vi "Convert and Enqueue.vi"(8 "error in":errorcluster, 10 "UI GUID":string, 11 "Data":u8[](array[numeric])) -> (0 "error out":errorcluster, 3 "Table Data":string[][](array[string]))   [LabVIEW 2025, in "CAN-LIN Raw Bus Capture UI.lvlib"]
uses:
  CAN-LIN Raw Bus Capture UI.lvlib
  Enqueue Data.vi
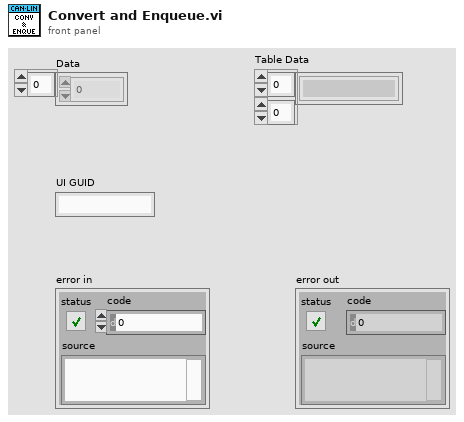
[diagram p1: front panel]
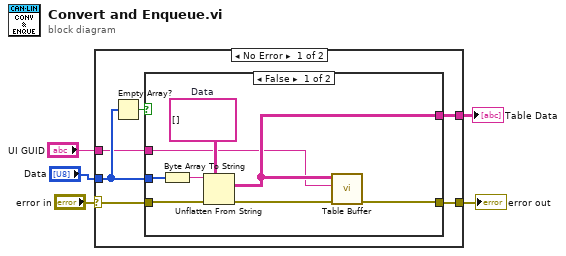
[diagram p0: block diagram]
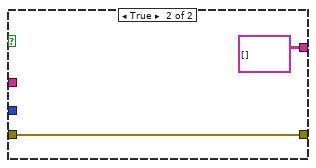
[diagram p2: hidden frame]
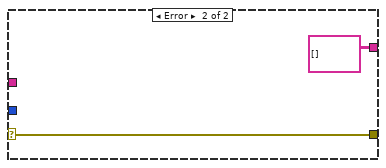
[diagram p3: hidden frame]
diagram:
  n1 = case shown="No Error" "error in" {
    selector: "error in" -> [w11 w23]
    tunnel: [w10 w23] -> w4
    tunnel: "Data" -> [w8 _]
    tunnel: [w7 string[][] [] ("Fetched I2C Messages")] -> w2
    tunnel: "UI GUID" -> [w6 _]
    frame No Error {
      n2 = Empty Array?(array=w8) -> (empty?=w9:bool)
      n3 = case shown="False" w9 {
        tunnel: w11 -> [w17 w21]
        tunnel: [w14 w21] -> w10
        tunnel: w8 -> [w19 _]
        tunnel: [w13 string[][] [] ("Fetched I2C Messages")] -> w7
        tunnel: w6 -> [w12 _]
        frame False {
          w16 = string[][] []  # Data
          n4 = Byte Array To String(unsigned byte array=w19) -> (string=w18:string)
          n5 = Unflatten From String(type=w16, binary string=w18, error in (no error)=w17) -> (value=w13:string[][], error out=w15:errorcluster)  [unwired: 2 in, 1 out]
          n6 = call-poly "Table Buffer.vi"("error in"=w15, "UI GUID"=w12, "Data"=w13) -> ("error out"=w14:errorcluster)  [unwired: 7 in, 1 out]
        }
        frame True {
        }
      }
    }
    frame Error {
    }
  }
  "error out" <- w4
  "Table Data" <- w2
